vi "RanLate_.vi"() -> ()   [LabVIEW 2017]
uses:
  <vilib>/Platform/TimedLoop/XDataNode/timing_clust.ctl
  <vilib>/Platform/TimedLoop/XDataNode/nitl_modes.ctl
  <vilib>/Platform/TimedLoop/XDataNode/wakeup.ctl
  SoftmotionClass/SoftmotionAxis/SoftmotionAxis.lvclass
  <vilib>/platform/TimedLoop/XDataNode/XDataNode.xnode
  <vilib>/Platform/TimedLoop/XDataNode/XDNodeRunTimeDep.lvlib
  <resource>/objmgr/nimotion.rc
panel:
  out "Array":dbl[](array[numeric])
  out "Execution times (us)":dbl[](graph)
  out "max value":dbl
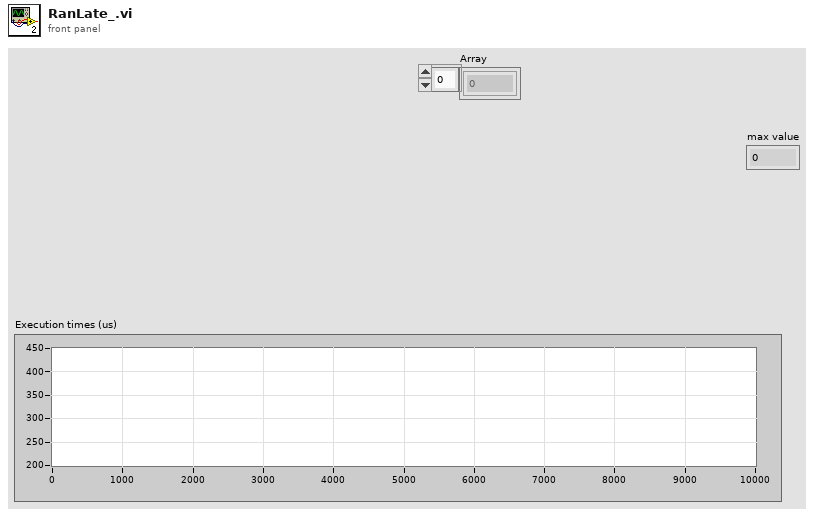
[diagram p1: front panel]
types:
  T1 = typedef "XDNodeRunTimeDep.lvlib/timing_clust.ctl" = cluster{"Expected End [f-1]":u64, "Actual End [f-1]":u64, "Finished Late? [f-1]":bool, "Expected End [i-1]":u64, "Actual End [i-1]":u64, "Finished Late? [i-1]":bool, "Expected Start [i]":u64, "Actual Start [i]":u64, "Expected Start [f]":u64, "Actual Start [f]":u64, "Source Name":string, "Structure Name":string, "Period":i64, "Deadline":i64, "Offset":i64, "Start":i64, "Priority":i32, "Timeout":i32, "Mode":T2, "Wakeup Reason":T3, "Error":errorcluster, "Source Type":string, "Secondary Source Type":string, "Global End Time":u64, "Global Start Time":u64, "Frame Duration":u64, "Iteration Duration":u64, "Assigned CPU":i32, "I/O Scan Engine Mode":u32}
  T2 = typedef "XDNodeRunTimeDep.lvlib/nitl_modes.ctl" = enum32{"No Change", "Process missed periods, maintain original phase", "Discard missed periods, maintain original phase", "Process missed periods, ignore original phase", "Discard missed periods, ignore original phase"}
  T3 = typedef "XDNodeRunTimeDep.lvlib/wakeup.ctl" = enum32{"Normal", "Aborted", "Asynchronous wakeup", "Timing source error", "Timed loop error", "Timeout"}
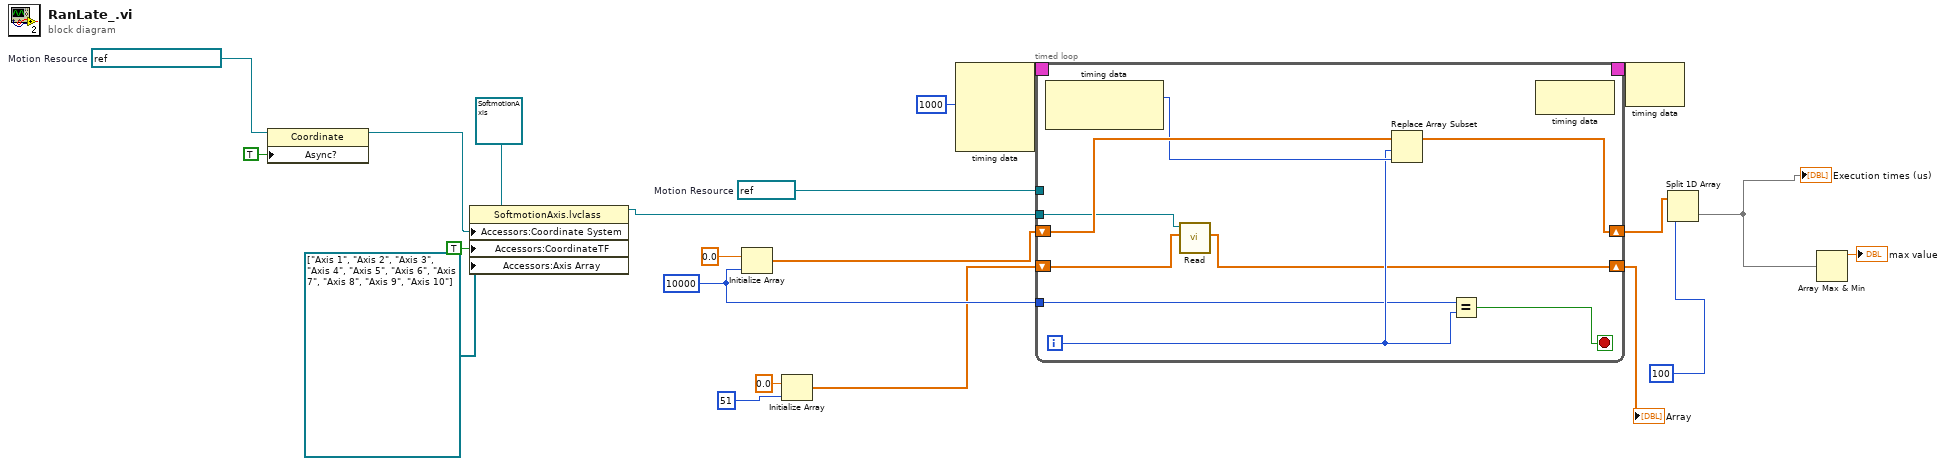
[diagram p0: block diagram]
diagram:
  w2 = refnum<k21> "Coordinate Space 1"  # Motion Resource
  w16 = 10000 ("dimension size")
  w20 = refnum<k21> "Axis 1"  # Motion Resource
  n1 = property class="Coordinate"(reference=w2, "Async?"=TRUE) -> (reference out=w1:refnum<k21>)  [unwired: 1 in, 1 out]
  n2 = property class="SoftmotionAxis.lvclass"(reference=refnum<class "SoftmotionAxis.lvclass"> refnum ("SoftmotionAxis.lvclass"), "Accessors:Coordinate System"=w1, "Accessors:CoordinateTF"=TRUE ("CoordinateTF"), "Accessors:Axis Array"=refnum<k21>[] ["Axis 1", "Axis 2", "Axis 3", "Axis 4", "Axis 5", "Axis 6", "Axis 7", "Axis 8", "Axis 9", "Axis 10"] ("Axis Array")) -> (reference out=w8:refnum<class "SoftmotionAxis.lvclass">)  [unwired: 1 in, 1 out]
  n3 = Initialize Array(0.0 ("element"), w16) -> (w17:dbl[])
  n4 = Initialize Array(0.0 ("element"), 51 ("dimension size")) -> (w5:dbl[])
  n5 = node-c288(i64 1000 ("Period")) -> (w22:T1)  [unwired: 3 in]
  n6 = timed-loop {
    timing: w22 -> [_]
    timing-out: [_] -> w21
    tunnel: w20 -> [_]
    shift-right: [w29] -> w14
    shift-left: w17 -> [w31]
    tunnel: w16 -> [w27]
    tunnel: w8 -> [w25]
    shift-right: [w24] -> w4
    shift-left: w5 -> [w23]
    i -> [w28]
    stop <- w26 stop-if-true
    n7 = node-c288() -> (w30:i64)  [unwired: 1 in, 1 out]
    n8 = call-dynamic "Read.vi"("Results Array In"=w23, "SoftmotionAxis in"=w25) -> ("appended array"=w24:dbl[])  [unwired: 7 in, 2 out]
    n9 = Replace Array Subset(array=w31, new element=w30, index=w28) -> (w29:dbl[])
    n10 = Equal?(x=w27, y=w28) -> (x = y?=w26:bool)
    n11 = node-c288() -> ()  [unwired: 1 in, 1 out]
  }
  "Array" <- w4
  n12 = node-c288(w21) -> ()  [unwired: 1 out]
  n13 = Split 1D Array(array=w14, index=100) -> (second subarray=w12:dbl[])  [unwired: 1 out]
  "Execution times (us)" <- w12
  n14 = Array Max & Min(array=w12) -> (max value=→"max value":dbl)  [unwired: 3 out]
